vi "Delete Entry.vi"(7 "Time Entry Store in":refnum<class "Time Entry Store-INI.lvclass">, 8 "error in (no error)":errorcluster, 10 "Start Time":timestamp, 11 "ID":string) -> (0 "error out":errorcluster, 3 "found?":bool, 5 "Time Entry Store out":refnum<class "Time Entry Store-INI.lvclass">)   [LabVIEW 2024, in "Time Entry Store-INI.lvclass"]
doc: "Deletes the time entry with the given ID from the month file of Start Time (UTC) and rewrites that file. found? is FALSE and nothing is written when the entry is not there.\n\nGenerated by: Claude"
uses:
  Time Entry Store-INI.lvclass
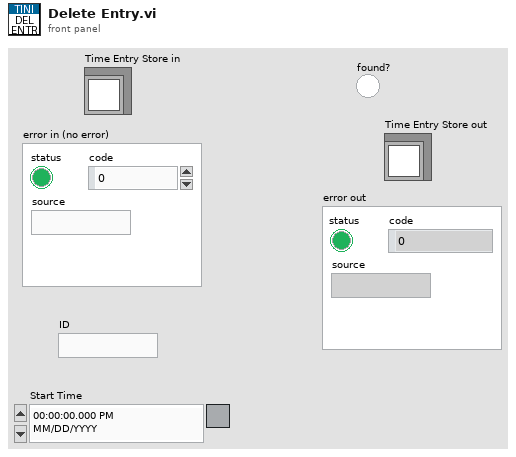
[diagram p1: front panel]
types:
  T1 = typedef "Time Entry List.ctl" = T2[]
  T2 = typedef "Time Entry.ctl" = cluster{"ID":string, "Project ID":string, "Task ID":string, "Start Time":timestamp, "End Time":timestamp, "Description":string}
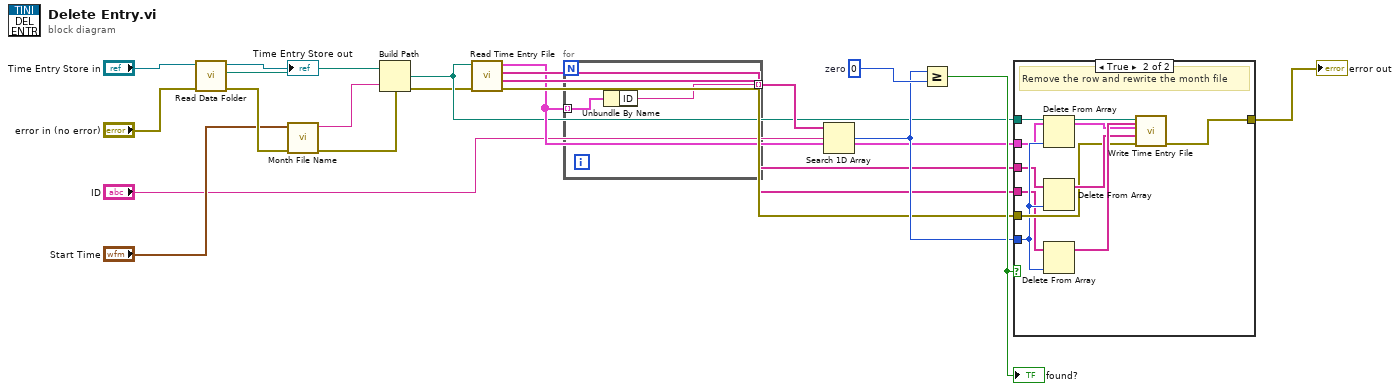
[diagram p0: block diagram]
diagram:
  w17 = 0  # zero
  n1 = call-dynamic "Read Data Folder.vi"("error in (no error)"="error in (no error)", "Time Entry Store-INI in"="Time Entry Store in") -> ("error out"=w5:errorcluster, "Data Folder"=w7:path, "Time Entry Store-INI out"=→"Time Entry Store out":refnum<class "Time Entry Store-INI.lvclass">)  [unwired: 7 in]
  n2 = call "Month File Name.vi"("error in (no error)"=w5, "Start Time"="Start Time") -> ("error out"=w9:errorcluster, "File Name"=w8:string)  [unwired: 8 in]
  n3 = Build Path(base path=w7, name or relative path=w8) -> (appended path=w10:path)
  n4 = call "Read Time Entry File.vi"("error in (no error)"=w9, "File Path"=w10) -> ("error out"=w14:errorcluster, "Task Names"=w13:string[], "Project Names"=w12:string[], "Time Entries"=w11:T1)  [unwired: 6 in]
  n5 = for {
    tunnel: w11 -> [w20] mode=indexing
    tunnel: [w21] -> w15 mode=indexing
    n6 = Unbundle By Name(w20) -> ("ID"=w21:string)
  }
  n7 = Search 1D Array(1D array=w15, element="ID") -> (index of element=w16:i32)  [unwired: 1 in]
  n8 = Greater Or Equal?(x=w16, y=w17) -> (x >= y?=w18:bool)
  "found?" <- w18
  n9 = case shown="True" w18 {
    tunnel: w10 -> [_ w23]
    tunnel: w11 -> [_ w24]
    tunnel: w12 -> [_ w25]
    tunnel: w13 -> [_ w26]
    tunnel: w14 -> [w22 w28]
    tunnel: w16 -> [_ w27]
    tunnel: [w22 w32] -> w19
    frame False {
      # "Not there - leave the file alone"
    }
    frame True {
      # "Remove the row and rewrite the month file"
      n10 = Delete From Array(array=w24, index=w27) -> (array with subset deleted=w29:T1)  [unwired: 1 in, 1 out]
      n11 = Delete From Array(array=w25, index=w27) -> (array with subset deleted=w30:string[])  [unwired: 1 in, 1 out]
      n12 = Delete From Array(array=w26, index=w27) -> (array with subset deleted=w31:string[])  [unwired: 1 in, 1 out]
      n13 = call "Write Time Entry File.vi"("Task Names"=w31, "error in (no error)"=w28, "Project Names"=w30, "Time Entries"=w29, "File Path"=w23) -> ("error out"=w32:errorcluster)  [unwired: 6 in]
    }
  }
  "error out" <- w19
